vi "Init Write Test.vi"(0 "interface":refnum<k21>, 1 "Intf.BaudRate64":u64, 2 "Intf.CAN.Term":u32, 3 "error in (no error)":errorcluster) -> (7 "session out":refnum<k21>, 10 "error out":errorcluster)   [LabVIEW 2023]
uses:
  <resource>/objmgr/xnet.rc
  <vilib>/xnet/xnet.llb/XNET Create Session (Signal Output Single-point).vi
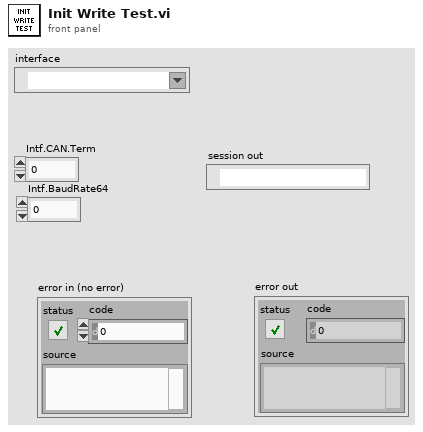
[diagram p1: front panel]
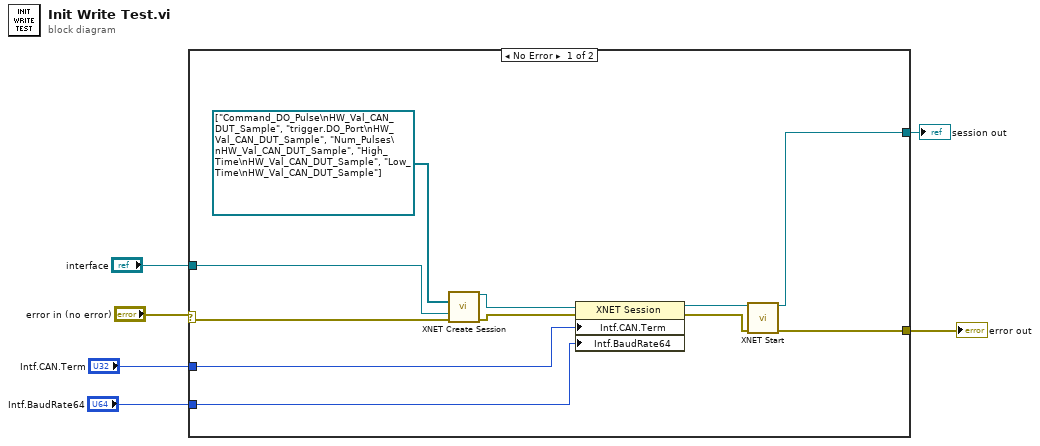
[diagram p0: block diagram]
diagram:
  n1 = case shown="No Error" "error in (no error)" {
    selector: "error in (no error)" -> [w16 w18]
    tunnel: "Intf.CAN.Term" -> [w13 _]
    tunnel: "Intf.BaudRate64" -> [w12 _]
    tunnel: [w9 w18] -> w3
    tunnel: [w10 _] -> w2
    tunnel: "interface" -> [w7 _]
    frame No Error {
      n2 = call-poly <vilib>:"XNET Create Session.vi"("signal list"=refnum<k21>[] ["Command_DO_Pulse\nHW_Val_CAN_DUT_Sample", "trigger.DO_Port\nHW_Val_CAN_DUT_Sample", "Num_Pulses\nHW_Val_CAN_DUT_Sample", "High_Time\nHW_Val_CAN_DUT_Sample", "Low_Time\nHW_Val_CAN_DUT_Sample"], "interface"=w7, "error in (no error)"=w16) -> ("session out"=w15:refnum<k21>, "error out"=w14:errorcluster)  [unwired: 11 in]
      n3 = property class="XNET Session"(reference=w15, error in=w14, "Intf.CAN.Term"=w13, "Intf.BaudRate64"=w12) -> (reference out=w11:refnum<k21>, error out=w8:errorcluster)
      n4 = call <vilib>:"XNET Start.vi"("session in"=w11, "error in (no error)"=w8) -> ("session out"=w10:refnum<k21>, "error out"=w9:errorcluster)  [unwired: 12 in]
    }
    frame Error {
    }
  }
  "error out" <- w3
  "session out" <- w2
